vi "drawLines.vi"(0 "reference":refnum<class "Graphics.lvclass">, 1 "points":T2[](array[typedef]) {"y" format="%.2f"; "x" format="%.2f"}, 2 "lineWidth(1)":dbl=1.0 format="%.2f", 3 "color(if not used=default color)":u32=536870912 format="%.0x", 4 "fill?(F)":bool, 5 "error in (no error)":errorcluster, 7 "stroke":T1) -> (14 "reference out":refnum<class "Graphics.lvclass">, 19 "error out":errorcluster)   [LabVIEW 2020, in "Graphics.lvclass"]
doc: "Draws lines\nIf point=(NaN,???), The pen will be lifted\nand start over from the next point (put down)."
uses:
  <resource>/Framework/Providers/Open_GDS/UML/Graphics_class/Graphics.lvclass
  <resource>/Framework/Providers/Open_GDS/UML/General/Point/Point Point2D.ctl
  <resource>/Framework/Providers/Open_GDS/UML/Graphics_class/StrokeType.ctl
panel:
  # "Always set\nVI Server class\nto current VI. Do not\nconnect this control\nto the connector pane.\n(Tip!: Just drag\nand drop the icon\ninto the refnum)"
  # "If point=(NaN,???), The pen will be lifted\nand start over from the next point (put down)."
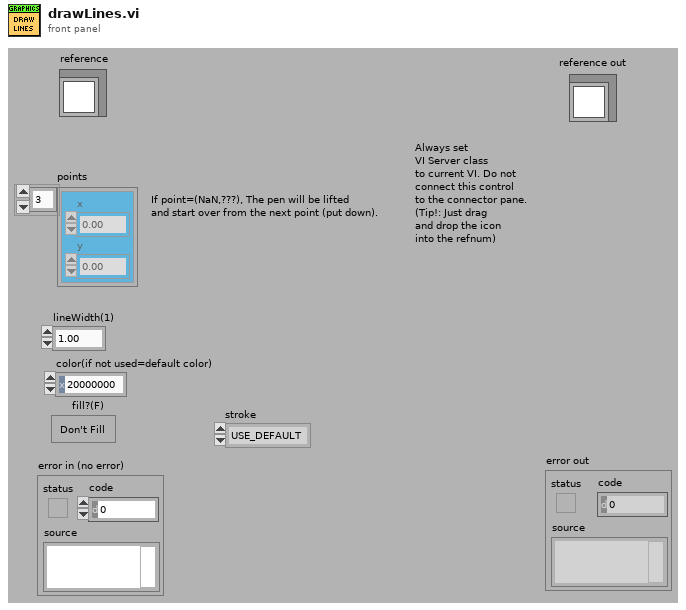
[diagram p1: front panel]
types:
  T1 = typedef "Graphics.lvclass/StrokeType.ctl" = enum16{"USE_DEFAULT", "SOLID", "DOTTED"}
  T2 = typedef "Point Point2D.ctl" = cluster{"x":dbl, "y":dbl}
  T3 = typedef "Graphics.lvclass/ObjectAttributes.ctl" = cluster{"drawColor":u32, "backgroundColor":u32, "font":T4, "fontType":T5, "picture":picture, "stroke":T1, "scaleX":dbl, "scaleY":dbl, "screenRef":refnum<vi>, "offsetX":dbl, "offsetY":dbl}
  T4 = typedef "Graphics.lvclass/FontType.ctl" = cluster{"Font Name:":string, "Size":i16, "Strikeout?":bool, "Italic?":bool, "Underline?":bool, "Outline?":bool, "Shadow?":bool, "Bold?":bool}
  T5 = typedef "Graphics.lvclass/LvFontType.ctl" = enum16{"User-specified Font", "Application Font", "System Font", "Dialog Font"}
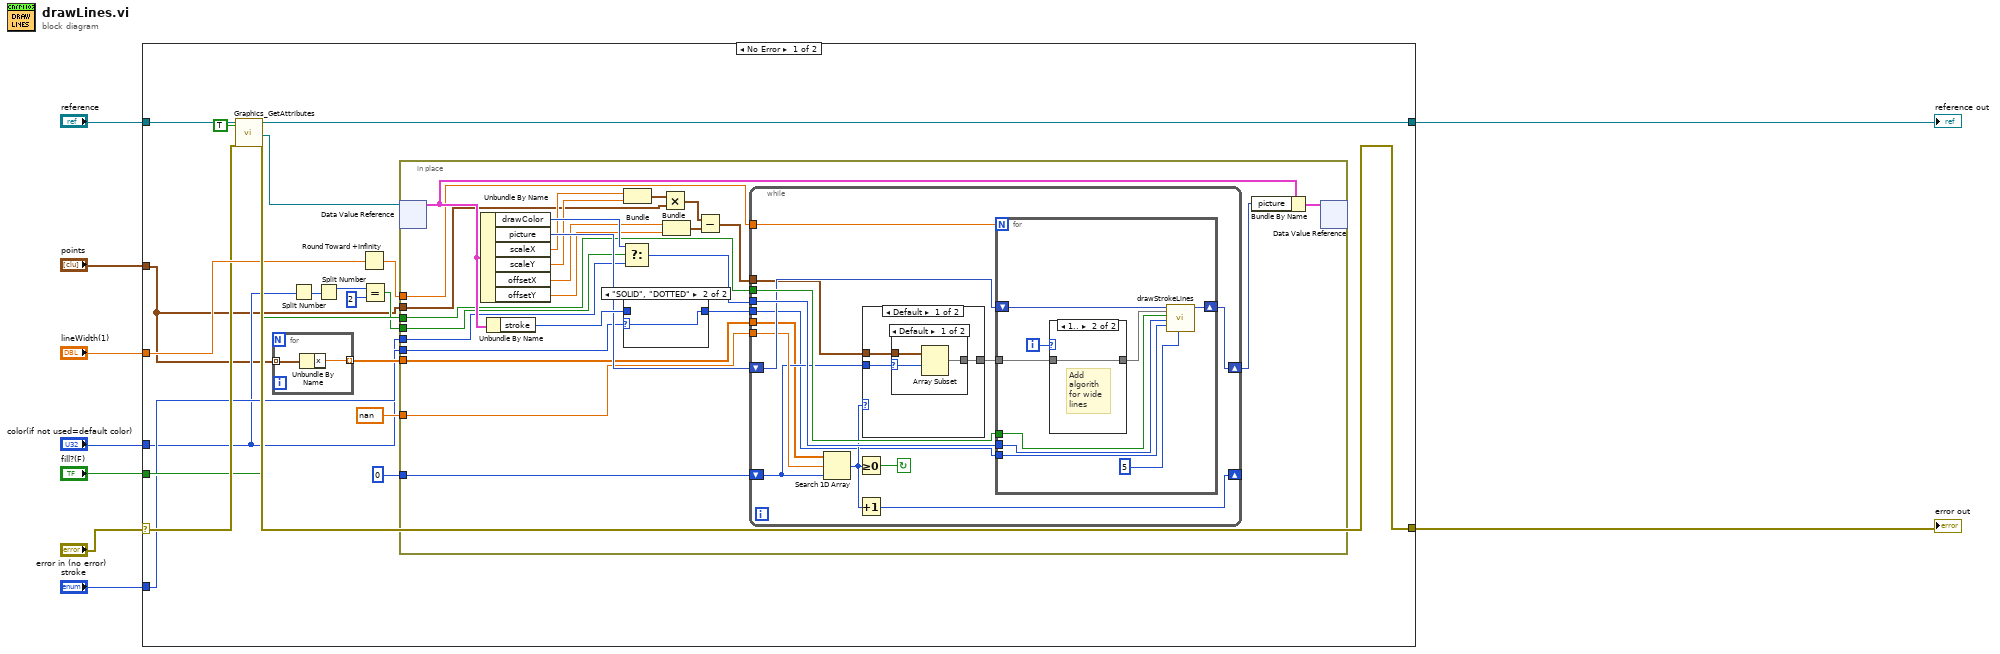
[diagram p0: block diagram]
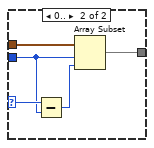
[diagram p4: hidden frame]
diagram:
  n1 = case shown="No Error" "error in (no error)" {
    selector: "error in (no error)" -> [w21 w95]
    tunnel: "reference" -> [w28 w96]
    tunnel: [w27 w95] -> w8
    tunnel: [w26 w96] -> w7
    tunnel: "points" -> [w10 _]
    tunnel: "lineWidth(1)" -> [w25 _]
    tunnel: "color(if not used=default color)" -> [w12 _]
    tunnel: "fill?(F)" -> [w17 _]
    tunnel: "stroke" -> [w13 _]
    frame No Error {
      n2 = call <resource>:"Graphics_GetAttributes.vi"("reference in"=w28, "OnlyGetDvrReference(False)"=TRUE, "error in (no error)"=w21) -> ("reference out"=w26:refnum<class "Graphics.lvclass">, "DataRef"=w19:refnum<data-value>, "error out"=w27:errorcluster)  [unwired: 13 in, 1 out]
      n3 = for {
        tunnel: w10 -> [w94] mode=indexing
        tunnel: [w93] -> w14 mode=indexing
        n4 = Unbundle By Name(w94) -> ("x"=w93:dbl)
      }
      n5 = Split Number(x=w12) -> (hi(x)=w24:u16)  [unwired: 1 out]
      n6 = Split Number(x=w24) -> (hi(x)=w23:u8)  [unwired: 1 out]
      n7 = Round Toward +Infinity(x=w25) -> (ceil(x): smallest int >= x=w18:dbl)
      n8 = Equal?(x=w23, y=u8 2) -> (x = y?=w11:bool)
      n9 = in-place {
        in-place-border: w18 -> [w42]
        in-place-border: w17 -> [w40]
        in-place-border: 0 -> [w39]
        in-place-border: nan -> [w38]
        in-place-border: w14 -> [w37]
        in-place-border: w13 -> [w35]
        in-place-border: w12 -> [w34]
        in-place-border: w11 -> [w33]
        in-place-border: w10 -> [w29]
        n10 = in-place-dvr #1(w19) -> (w53:T3)  [unwired: 1 out]
        n11 = Unbundle By Name(w53) -> ("drawColor"=w49:u32, "picture"=w48:picture, "scaleX"=w47:dbl, "scaleY"=w46:dbl, "offsetX"=w45:dbl, "offsetY"=w44:dbl)
        n12 = Unbundle By Name(w53) -> ("stroke"=w50:T1)
        n13 = Select(t=w49, s=w33, f=w34) -> (s? t:f=w41:u32)
        n14 = Bundle("scaleX"=w47, "scaleY"=w46) -> (w32:cluster{"scaleX":dbl, "scaleY":dbl})  [unwired: 1 out]
        n15 = case shown="\"SOLID\", \"DOTTED\"" w35 {
          selector: w35 -> [_ w55]
          tunnel: [w54 w55] -> w36
          tunnel: w50 -> [w54 _]
          frame "USE_DEFAULT", Default {
          }
          frame "SOLID", "DOTTED" {
          }
        }
        n16 = Multiply(x=w32, y=w29) -> (x*y=w30:T2[])
        n17 = Bundle("offsetX"=w45, "offsetY"=w44) -> (w31:cluster{"offsetX":dbl, "offsetY":dbl})  [unwired: 1 out]
        n18 = Subtract(x=w30, y=w31) -> (x-y=w43:T2[])
        n19 = while {
          tunnel: w43 -> [w58]
          tunnel: w42 -> [w69]
          tunnel: w41 -> [w68]
          tunnel: w40 -> [w67]
          shift-right: [w65] -> w52
          shift-left: w48 -> [w66]
          shift-right: [w64] -> _
          shift-left: w39 -> [w59]
          tunnel: w38 -> [w63]
          tunnel: w37 -> [w57]
          tunnel: w36 -> [w56]
          stop <- w60 continue-if-true
          n20 = Search 1D Array(1D array=w57, element=w63, start index (0)=w59) -> (index of element=w61:i32)
          n21 = Greater Or Equal To 0?(x=w61) -> (x >= 0?=w60:bool)
          n22 = Increment(x=w61) -> (x+1=w64:i32)
          n23 = case shown="Default" w61 {
            selector: w61 -> [_ w78]
            tunnel: w58 -> [w71 w81]
            tunnel: [w70 w80] -> w62
            tunnel: w59 -> [w72 w77]
            frame Default {
              n24 = case shown="Default" w72 {
                selector: w72 -> [w73 _]
                tunnel: w71 -> [w75 w76]
                tunnel: [w74 w76] -> w70
                frame Default {
                  n25 = Array Subset(array=w75, index=w73) -> (w74:T2[])  [unwired: 1 in]
                }
                frame 0 {
                }
              }
            }
            frame 0.. {
              n26 = Subtract(x=w78, y=w77) -> (x-y=w79:i32)
              n27 = Array Subset(array=w81, index=w77, length=w79) -> (w80:T2[])
            }
          }
          n28 = for {
            N: w69 -> [_]
            tunnel: w62 -> [w88]
            tunnel: w68 -> [w89]
            shift-right: [w84] -> w65
            shift-left: w66 -> [w90]
            tunnel: w67 -> [w85]
            tunnel: w56 -> [w83]
            i -> [w87]
            n29 = case shown="1.." w87 {
              tunnel: [w91 w92] -> w86
              tunnel: w88 -> [w91 w92]
              frame 0, Default {
              }
              frame 1.. {
                # "Add algorith for wide lines"
              }
            }
            n30 = call <resource>:"drawStrokeLines.vi"("picture"=w90, "line endpoints"=w86, "fill?(F)"=w85, "color(black)"=w89, "stroke"=w83, "strokeLength"=5) -> ("new picture"=w84:picture)  [unwired: 2 in, 11 out]
          }
        }
        n31 = Bundle By Name(cluster=w53, "picture"=w52) -> (w51:T3)
        n32 = in-place-dvr #1(w51) -> ()  [unwired: 2 out]
      }
    }
    frame Error {
    }
  }
  "reference out" <- w7
  "error out" <- w8
